vi "Documentation.vi"() -> (0 "Author":string, 1 "History":string, 2 "Version":string, 3 "Description":string)   [LabVIEW 2021, in "CAN_Reader_CANsub_Plugin.lvlib"]
uses:
  CAN_Reader_CANsub_Plugin.lvlib
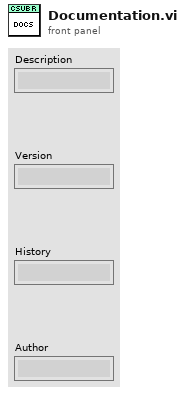
[diagram p1: front panel]
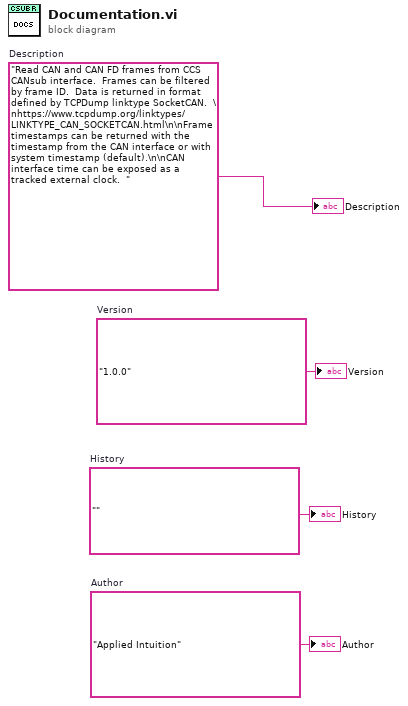
[diagram p0: block diagram]
diagram:
  w1 = "Applied Intuition"  # Author
  w2 = ""  # History
  w3 = "1.0.0"  # Version
  w4 = "Read CAN and CAN FD frames from CCS CANsub interface.  Frames can be filtered by frame ID.  Data is returned in format defined by TCPDump linktype SocketCAN.  \nhttps://www.tcpdump.org/linktypes/LINKTYPE_CAN_SOCKETCAN.html\n\nFrame timestamps can be returned with the timestamp from the CAN interface or with system timestamp (default).\n\nCAN interface time can be exposed as a tracked external clock.  "  # Description
  "Description" <- w4
  "Version" <- w3
  "History" <- w2
  "Author" <- w1
